vi "Cleanup Device.vi"(8 "error in (no error)":errorcluster, 11 "Device in":refnum<class "Device.lvclass">) -> (0 "error out":errorcluster, 3 "Device out":refnum<class "Device.lvclass">)   [LabVIEW 2020, in "HAL.lvlib" / "Device.lvclass"]
doc: "This VI should be overridden primarly for By Reference implementation of devices, usually to delete a DVR. Anything else that is allocated or setup in the Ctor VI should be undone in cleanup. After this VI runs the class instance will no longer be available for opening."
uses:
  Device.lvclass
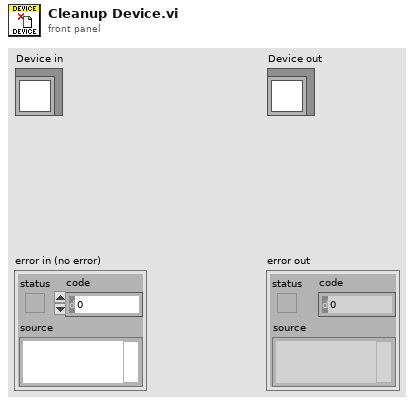
[diagram p1: front panel]
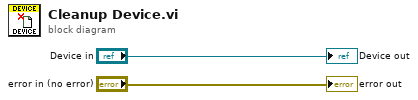
[diagram p0: block diagram]
diagram:
  "error out" <- "error in (no error)"
  "Device out" <- "Device in"
